vi "I2C Read Reg 16.vi"(8 "error in (no error)":errorcluster, 11 "I2C Device":T1) -> (0 "error out":errorcluster, 2 "Value":u16, 3 "I2C Device out":T1)   [LabVIEW 2020, in "wiringPi.lvlib"]
doc: "<b>_______________________________________________________________</b>\n** Author: Juan José Villacorta\n** LabVIEW wrapper for C library <b> wiringPi </b>,\n** https://github.com/WiringPi/WiringPi\n<b>_______________________________________________________________</b>\n/*\n * Read an 16-bit value from a register on the device\n**********************************************************************************\n*/"
uses:
  wiringPi.lvlib
  Type Defs/I2C Device.ctl
panel:
  in  "Register":i32
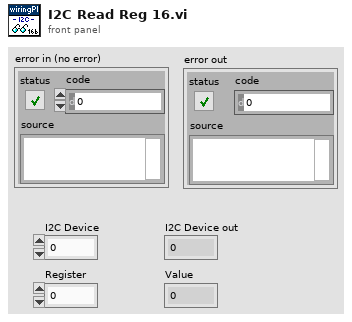
[diagram p1: front panel]
types:
  T1 = typedef "wiringPi.lvlib/I2C Device.ctl" = i32
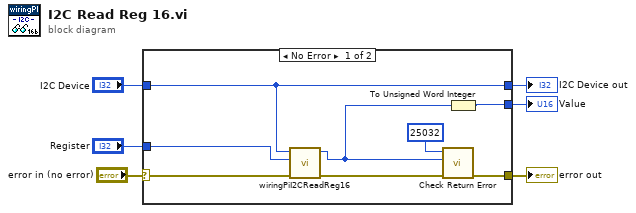
[diagram p0: block diagram]
diagram:
  n1 = case shown="No Error" "error in (no error)" {
    selector: "error in (no error)" -> [w13 w16]
    tunnel: [w14 w16] -> w5
    tunnel: "I2C Device" -> [w11 w15]
    tunnel: [w11 w15] -> w4
    tunnel: [w8 _] -> w3
    tunnel: "Register" -> [w7 _]
    frame No Error {
      n2 = call "wiringPiI2CReadReg16.vi"("error in (no error)"=w13, "reg"=w7, "devID"=w11) -> ("error out"=w12:errorcluster, "return"=w10:i32)  [unwired: 7 in]
      n3 = call "Check Return Error.vi"("error in (no error)"=w12, "Return code"=w10, "Error number"=25032) -> ("error out"=w14:errorcluster)  [unwired: 8 in]
      n4 = To Unsigned Word Integer(number=w10) -> (unsigned 16bit integer=w8:u16)
    }
    frame Error {
    }
  }
  "error out" <- w5
  "I2C Device out" <- w4
  "Value" <- w3
